vi "write_Float.vi"(8 "错误输入（无错误）":errorcluster, 9 "Value":dbl, 10 "Address":string, 11 "URL":string="opc://localhost/National Instruments.NIOPCServers.V5/Channel1.Battery_Testing.") -> (0 "error out":errorcluster caption="错误输出", 3 "ok?":bool)   [LabVIEW 2013]
panel:
  out "数据":u16
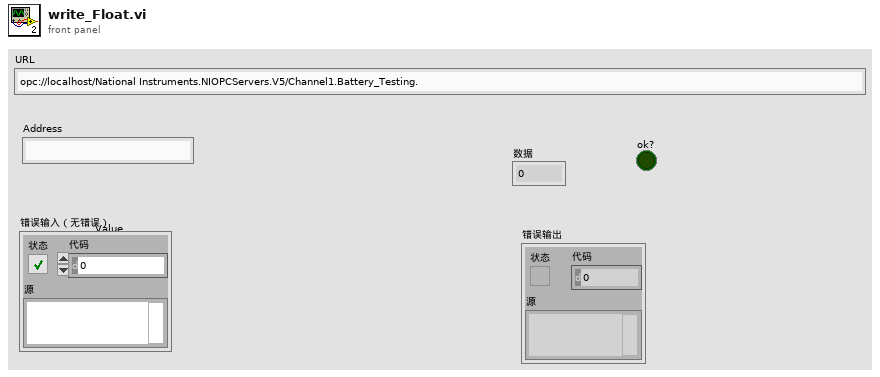
[diagram p1: front panel]
types:
  T1 = enum16{"Read", "Write", "ReadWrite", "BufferedRead", "BufferedReadWrite"}
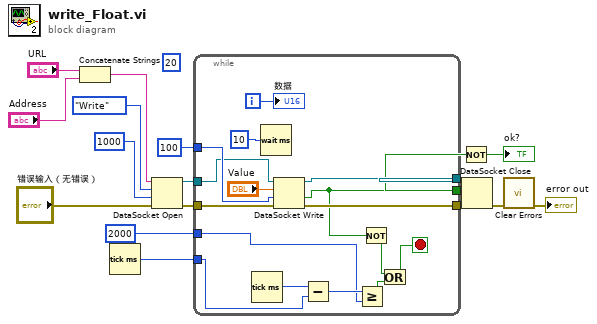
[diagram p0: block diagram]
diagram:
  (unwired) 20
  n1 = Concatenate Strings("URL", "Address") -> (w15:string)
  n2 = Tick Count (ms)() -> (millisecond timer value=w1:u32)
  n3 = DataSocket Open(8:"错误输入（无错误）", 9:1000 ("毫秒超时(10000)"), 10:T1."Write" ("模式"), 11:w15) -> (0:w11:errorcluster, 3:w10:refnum<k13>)
  n4 = while {
    tunnel: 100 ("毫秒超时(0)") -> [w32]
    tunnel: w11 -> [w31]
    tunnel: w10 -> [w30]
    tunnel: [w29] -> w9
    tunnel: [w28] -> w8
    tunnel: [w19] -> w5
    tunnel: 2000 ("毫秒超时(0)") -> [w21]
    tunnel: w1 -> [w20]
    i -> [w26]
    stop <- w22 stop-if-true
    n5 = Tick Count (ms)() -> (millisecond timer value=w23:u32)
    n6 = Wait (ms)(milliseconds to wait=u32 10 ("等待时间（毫秒）")) -> ()  [unwired: 1 out]
    n7 = DataSocket Write(8:w31, 9:w32, 10:"Value", 11:w30) -> (0:w28:errorcluster, 1:w19:bool, 3:w29:refnum<k13>)
    n8 = Subtract(x=w23, y=w20) -> (x-y=w24:u32)
    n9 = Greater Or Equal?(x=w24, y=w21) -> (x >= y?=w25:bool)
    n10 = Not(x=w19) -> (.not. x?=w18:bool)
    n11 = Or(x=w18, y=w25) -> (x .or. y?=w22:bool)
    "数据" <- w26
  }
  n12 = Not(x=w5) -> (.not. x?=→"ok?":bool)
  n13 = DataSocket Close(8:w8, 11:w9) -> (0:w7:errorcluster)  [unwired: 1 in, 1 out]
  n14 = call <vilib>:"Clear Errors.vi"("error in (no error)"=w7) -> ("error out"=→"error out":errorcluster)  [unwired: 6 in]
